vi "SMTP Email Send Text Message.vi"(0 "smtp session":T1 caption="session smtp", 2 "return address":string caption="adresse de retour", 3 "character set":string caption="jeu de caractères", 5 "recipients":string[](array[string]) caption="destinataires", 7 "subject":string caption="objet", 9 "message":string, 11 "error in (no error)":errorcluster caption="entrée d'erreur (pas d'erreur)", 12 "translit":string) -> (4 "smtp session out":T1 caption="session smtp en sortie", 6 "invalid recipients":string[](array[string]) caption="destinataires non valides", 15 "error out":errorcluster caption="sortie d'erreur")   [LabVIEW 2022 SP3, in "Copie de NI_SMTPEmail.lvlib"]
doc: "Envoie par e-mail le message textuel vers les destinataires en utilisant Mailserver.\n\nMessage textuel : Message textuel à envoyer; S'il n'y en a pas alors seules les pièces jointes seront envoyées.\n\nMailserver : Mailserver SMTP à utiliser pour envoyer le mail. Doit être spécifié ici ou configuré en utilisant SMTP Setup.vi\n\nAdresse de retour : l'adresse de retour de votre choix ; elle peut être spécifiée ici ou configurée en utilisant SMTP Setup.vi\n\nDestinataires : liste des adresses e-mail vers où envoyer votre e-mail.\n\nObjet : objet de votre message. \"Aucune\" est la chaîne par défaut si l'entrée n'est pas câblée.\n\nJeu de caractères : la messagerie fournit un support international. La valeur de jeu de caractères est nécessaire pour fonctionner avec les jeux de caractères étrangers (non-US).\n\nDestinataires non valides : la liste des destinataires (hormis ceux spécifiés) qui n'existent pas selon le serveur mail (qui peut très bien ne pas contenir tous les destinataires non valides, surtout s'ils ne sont pas locaux pour le serveur SMTP)."
uses:
  Copie de NI_SMTPEmail.lvlib
  SMTP Email Session.ctl
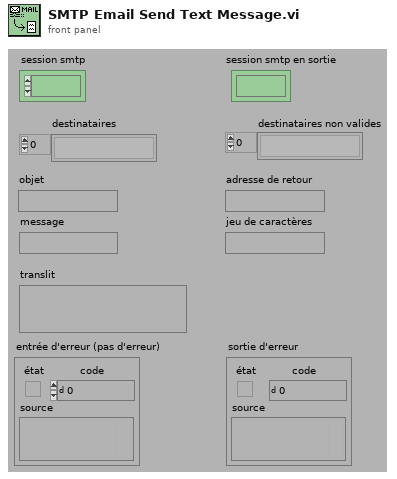
[diagram p1: front panel]
types:
  T1 = typedef "Copie de NI_SMTPEmail.lvlib/SMTP Email Session.ctl" = refnum<k1>
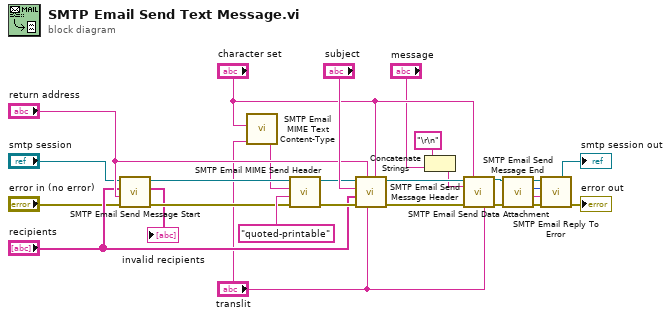
[diagram p0: block diagram]
diagram:
  n1 = call "SMTP Email Send Message Start.vi"("error in (no error)"="error in (no error)", "return address"="return address", "recipients"="recipients", "smtp session"="smtp session") -> ("error out"=w16:errorcluster, "invalid recipients"=→"invalid recipients":string[], "smtp session out"=w15:T1)  [unwired: 1 in]
  n2 = call "SMTP Email MIME Text Content-Type.vi"("translit"="translit", "character set"="character set") -> ("MIME content-type"=w2:string)  [unwired: 5 in]
  n3 = call "SMTP Email MIME Send Header.vi"("error in (no error)"=w16, "MIME content-transfer-encoding (7bit)"="quoted-printable" ("Content-Transfer-Encoding (\"7bit\")"), "MIME content-type (multipart/mixed)"=w2, "smtp session"=w15) -> ("error out"=w21:errorcluster, "smtp session out"=w22:T1)  [unwired: 2 in]
  n4 = call "SMTP Email Send Message Header.vi"("character set"="character set", "translit"="translit", "return address"="return address", "error in (no error)"=w21, "recipients"="recipients", "subject"="subject", "smtp session"=w22) -> ("error out"=w23:errorcluster, "smtp session out"=w24:T1)  [unwired: 3 in]
  n5 = Concatenate Strings("\r\n" ("Substring"), "message") -> (w4:string)
  n6 = call "SMTP Email Send Data Attachment.vi"("smtp session"=w24, "character set"="character set", "data"=w4, "error in (no error)"=w23, "translit"="translit") -> ("smtp session out"=w27:T1, "error out"=w26:errorcluster)  [unwired: 9 in]
  n7 = call "SMTP Email Send Message End.vi"("error in (no error)"=w26, "smtp session"=w27) -> ("error out"=w11:errorcluster, "reply"=w6:string, "reply code"=w7:i32, "smtp session out"=w10:T1)  [unwired: 2 in]
  n8 = call "SMTP Email Reply To Error.vi"("error in (no error)"=w11, "reply string in"=w6, "reply code in"=w7, "smtp session"=w10) -> ("error out"=→"error out":errorcluster, "smtp session out"=→"smtp session out":T1)  [unwired: 2 out]
